vi "PicoScope4000aUnitInfo.vi"(6 "error in (no error)":errorcluster, 8 "Mode":u16(ring) items=["Dialog On Error", "no dialog - CloseUnit and Stop", "no dialog - Continue", "no dialog - Stop"], 9 "handle in":i16) -> (0 "error out":errorcluster, 1 "Unit Info":T1, 2 "requiredSize":i16, 3 "handle out":i16)   [LabVIEW 2010]
uses:
  ps4000a.dll
panel:
  out "PICO_STATUS":u32
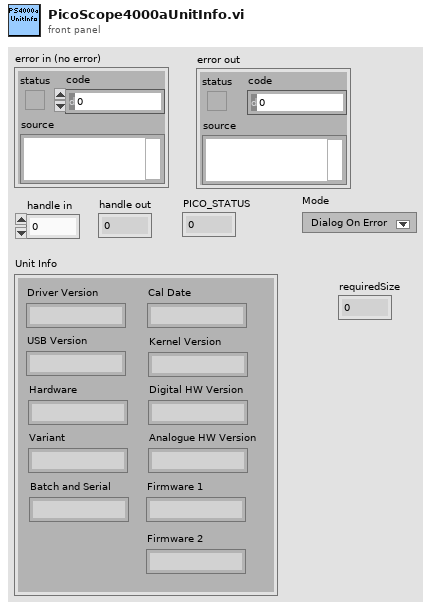
[diagram p1: front panel]
types:
  T1 = cluster{"Driver Version":string, "USB Version":string, "Hardware":string, "Variant":string, "Batch and Serial":string, "Cal Date":string, "Kernel Version":string, "Digital HW Version":string, "Analogue HW Version":string, "Firmware 1":string, "Firmware 2":string}
  T2 = cluster{"status":bool, "code":u32, "source":string}
  T3 = cluster{"[0]":string, "[1]":string, "[2]":string, "[3]":string, "[4]":string, "[5]":string, "[6]":string, "[7]":string, "[8]":string, "[9]":string, "[10]":string}
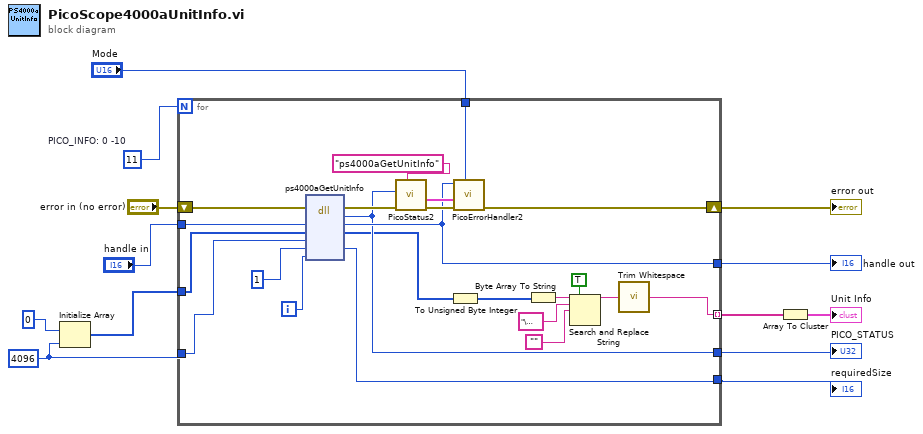
[diagram p0: block diagram]
diagram:
  w2 = i16 4096 ("requiredSize")
  w12 = 11  # PICO_INFO: 0 -10
  n1 = Initialize Array(i8 0 ("element"), w2) -> (w3:i8[])
  n2 = for {
    N: w12 -> [_]
    tunnel: "handle in" -> [w36]
    tunnel: [w19] -> w8 mode=indexing
    tunnel: [w27] -> w10
    tunnel: [w26] -> w9
    shift-right: [w28] -> w6
    shift-left: "error in (no error)" -> [w33]
    tunnel: "Mode" -> [w25]
    tunnel: w3 -> [w18]
    tunnel: w2 -> [w17]
    tunnel: [w14] -> w1
    i -> [w34]
    n3 = dll-call lib="ps4000A.dll" fn="ps4000aGetUnitInfo"(error in=w33, "handle"=w36, "unitInfo"=w18, "stringLength"=w17, "requiredSize"=i16 1 ("stringLength"), "pico_info"=w34) -> (error out=w31:errorcluster, "PICO_STATUS"=w26:u32, "handle"=w27:i16, "unitInfo"=w15:i8[], "requiredSize"=w14:i16)  [unwired: 4 in, 1 out]
    n4 = call "PicoStatus2.vi"("PICO source"="ps4000aGetUnitInfo" ("source"), "Error in"=w31, "PICO STATUS"=w26) -> ("error out"=w29:errorcluster, "PICO_STATUS out"=w30:T2)  [unwired: 5 in]
    n5 = To Unsigned Byte Integer(number=w15) -> (unsigned 8bit integer=w16:u8[])
    n6 = call "PicoErrorHandler2.vi"("Mode"=w25, "error in (no error)"=w29, "PICO_STATUS in"=w30, "handle In"=w27) -> ("error out"=w28:errorcluster)  [unwired: 7 in]
    n7 = Byte Array To String(unsigned byte array=w16) -> (string=w23:string)
    n8 = Search and Replace String(replace all?=TRUE ("replace all? (F)"), input string=w23, search string="\u0000", replace string="") -> (result string=w22:string)  [unwired: 4 in, 3 out]
    n9 = call <vilib>:"Trim Whitespace.vi"("string"=w22) -> ("trimmed string"=w19:string)  [unwired: 1 in]
  }
  "error out" <- w6
  "handle out" <- w10
  "PICO_STATUS" <- w9
  "requiredSize" <- w1
  n10 = Array To Cluster(array=w8) -> (cluster=→"Unit Info":T3)
